vi "Send HTTP request (custom).vi"(6 "value":string, 8 "error in (no error)":errorcluster, 9 "header":string, 10 "request":string, 11 "method":string="POST") -> (0 "error out":errorcluster, 1 "response":string, 2 "headers":string, 3 "status code":i32)   [LabVIEW 2020, in "MCP Server tests.lvlib"]
doc: "Test helper. Sends one HTTP request to the MCP test server at http://localhost:36987/mcp/server and returns the numeric HTTP status code, the raw response headers and the response body.\n\nmethod selects the HTTP method: GET and DELETE send no body, anything else is sent as POST with request as body. A Content-Type: application/json header is always sent. header and value add one extra request header, an empty header name adds none.\n\nstatus code is parsed from the status line at the start of headers and is 0 when no status line was received."
uses:
  MCP Server tests.lvlib
  <vilib>/httpClient/POSTBuffer.vi
  <vilib>/httpClient/LabVIEWHTTPClient.lvlib
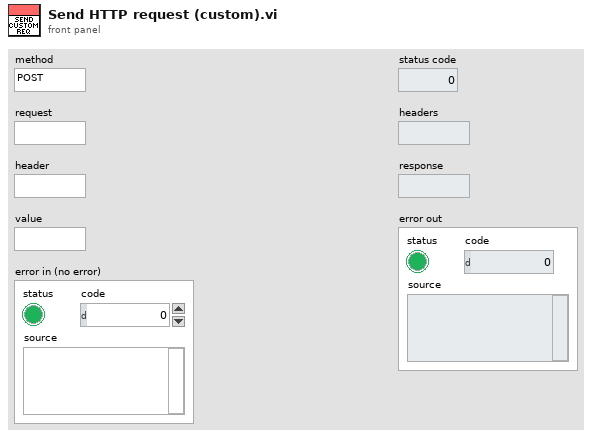
[diagram p1: front panel]
types:
  T1 = typedef "LabVIEWHTTPClient.lvlib/ClientHandle.ctl" = refnum<k1>
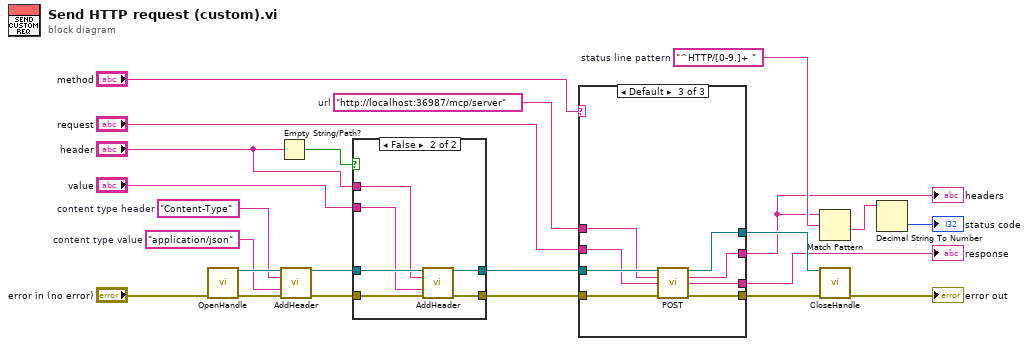
[diagram p0: block diagram]
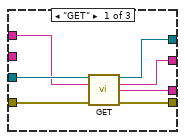
[diagram p2: hidden frame]
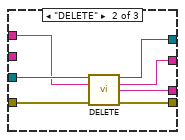
[diagram p3: hidden frame]
diagram:
  w6 = "^HTTP/[0-9.]+ "  # status line pattern
  w20 = "application/json"  # content type value
  w21 = "Content-Type"  # content type header
  w11 = "http://localhost:36987/mcp/server"  # url
  n1 = call <vilib>:"OpenHandle.vi"("error in (no error)"="error in (no error)") -> ("client handle out"=w22:T1, "error out"=w19:errorcluster)  [unwired: 13 in]
  n2 = Empty String/Path?(string/path="header") -> (empty?=w14:bool)
  n3 = call <vilib>:"AddHeader.vi"("client handle"=w22, "header"=w21, "value"=w20, "error in (no error)"=w19) -> ("client handle out"=w18:T1, "error out"=w17:errorcluster)  [unwired: 10 in]
  n4 = case shown="False" w14 {
    tunnel: w18 -> [w25 w31]
    tunnel: w17 -> [w24 w28]
    tunnel: "header" -> [_ w30]
    tunnel: "value" -> [_ w29]
    tunnel: [w25 w27] -> w13
    tunnel: [w24 w26] -> w12
    frame True {
    }
    frame False {
      n5 = call <vilib>:"AddHeader.vi"("client handle"=w31, "header"=w30, "value"=w29, "error in (no error)"=w28) -> ("client handle out"=w27:T1, "error out"=w26:errorcluster)  [unwired: 10 in]
    }
  }
  n6 = case shown="Default" "method" {
    tunnel: w13 -> [w38 w45 w53]
    tunnel: w12 -> [w36 w43 w50]
    tunnel: w11 -> [w37 w44 w52]
    tunnel: "request" -> [_ _ w51]
    tunnel: [w35 w42 w49] -> w8
    tunnel: [w34 w41 w48] -> w3
    tunnel: [w33 w40 w47] -> w2
    tunnel: [w32 w39 w46] -> w7
    frame "GET" {
      n7 = call <vilib>:"GET.vi"("client handle"=w38, "url"=w37, "error in (no error)"=w36) -> ("client handle out"=w35:T1, "headers"=w34:string, "body"=w33:string, "error out"=w32:errorcluster)  [unwired: 9 in]
    }
    frame "DELETE" {
      n8 = call <vilib>:"DELETE.vi"("client handle"=w45, "url"=w44, "error in (no error)"=w43) -> ("client handle out"=w42:T1, "headers"=w41:string, "body"=w40:string, "error out"=w39:errorcluster)  [unwired: 9 in]
    }
    frame Default {
      n9 = call-poly <vilib>:"POST.vi"("client handle"=w53, "url"=w52, "buffer"=w51, "error in (no error)"=w50) -> ("client handle out"=w49:T1, "headers"=w48:string, "body"=w47:string, "error out"=w46:errorcluster)  [unwired: 8 in]
    }
  }
  "headers" <- w3
  "response" <- w2
  n10 = Match Pattern(string=w3, regular expression=w6) -> (after substring=w5:string)  [unwired: 1 in, 3 out]
  n11 = call <vilib>:"CloseHandle.vi"("client handle"=w8, "error in (no error)"=w7) -> ("error out"=→"error out":errorcluster)  [unwired: 13 in]
  n12 = Decimal String To Number(string=w5) -> (number=→"status code":i32)  [unwired: 2 in, 1 out]
